vi "Process.vi"(8 "error in":errorcluster, 11 "Generator":refnum<class "Generator.lvclass">) -> (0 "error out":errorcluster, 3 "Generator out":refnum<class "Generator.lvclass">)   [LabVIEW 2019, in "Generator.lvclass"]
uses:
  Generator.lvclass
  <vilib>/JKI/JKI SMO/SMO/SMO.lvclass
  <userlib>/LevyLab/Debug/Debug.lvlib
  typedefs/Generator.State--enum.ctl
  929f499e-e52d-49ce-8fd4-6eb7de19c2ac.vi
  9c9ff3dc-a17c-4e79-91bb-522cf085dd97.vi
  7f9fb2fb-b452-4165-b08b-fdce49342378.vi
  C:/Program Files/National Instruments/LabVIEW 2019/vi.lib/JKI/JKI SMO/SMO/SMO.lvclass
panel:
  out "time (ms)":dbl=1.0 min=1.0 format="%#_6p"
  out "String 3":string
  in  "timeout (ms)":i32=10 min=1
  out "String 2":string
  out "String":string
  # "Generator"
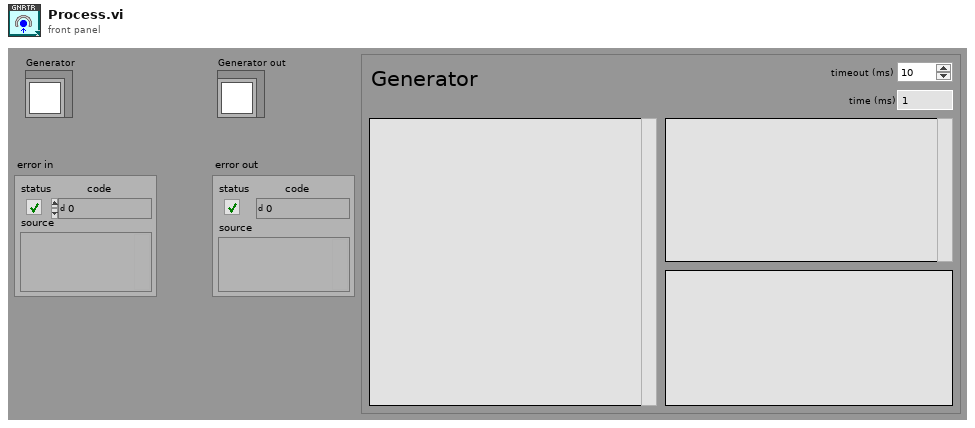
[diagram p1: front panel]
types:
  T1 = typedef "Generator.lvclass/Generator.State--enum.ctl" = enum16{"idle", "started"}
  T2 = enum32{"invalid app kind", "Development System", "Run Time System", "Student Edition", "Embedded LabVIEW", "Evaluation", "Custom"}
  T3 = enum32{"Invalid", "Standard", "Closed", "Hidden", "Minimized", "Maximized"}
  T4 = cluster{"Core":cluster{"Current VI Reference":refnum<vi>, "Close Panel on Exit?":bool, "Last Error":cluster{"error":errorcluster, "previous state":string, "remaining states":string}, "Shutdown?":bool}, "SelfRef":refnum<class "Generator.lvclass">, "state":T1}
  T5 = typedef "Generator.lvclass/AO.Channel--Cluster--Array.ctl" = T6[]
  T6 = typedef "Generator.lvclass/AO.Channel--Cluster.ctl" = cluster{"Enable?":bool, "Channel":i32, "Amplitude":dbl, "Offset":dbl, "Frequency":dbl, "Phase":dbl, "Function":T7, "Sweeping?":bool, "Limit AC?":bool, "Limit DC?":bool, "Duty Cycle?":bool, "Duty Cycle":dbl}
  T7 = typedef "Generator.lvclass/AO.Channel.Function--Enum.ctl" = enum16{"sine", "square", "triangle", "saw"}
  T8 = typedef "Generator.lvclass/REF.Channel--Cluster--Array.ctl" = T9[]
  T9 = typedef "Generator.lvclass/REF.Channel--Cluster.ctl" = cluster{"Enable?":bool, "Channel":i32, "Frequency":dbl, "Phase":dbl, "TC":dbl, "Roll-Off":i32}
  T10 = typedef "Generator.lvclass/Sweep.Channel--Cluster--Array.ctl" = T11[]
  T11 = typedef "Generator.lvclass/Sweep.Channel--Cluster.ctl" = cluster{"Enable?":bool, "Channel":u16, "Start":dbl, "End":dbl, "Pattern":T12, "Table":dbl[]}
  T12 = typedef "Generator.lvclass/Sweep.Pattern--Enum.ctl" = enum16{"Ramp /", "Ramp /\\", "Smooth Ramp _/", "Smooth Ramp _/\\_", "Table"}
  T13 = typedef "Generator.lvclass/Generator.Command--enum.ctl" = enum16{"start", "stop", "start sweep", "stop sweep"}
  T14 = cluster{"Current VI Reference":refnum<vi>, "Close Panel on Exit?":bool, "Last Error":cluster{"error":errorcluster, "previous state":string, "remaining states":string}, "Shutdown?":bool}
  T15 = typedef "Debug.lvlib/Attribute.Debug.lvclass/DebugBehavior.ctl" = enum16{"Normal", "Debug"}
  T16 = typedef "SMO.lvclass/Protected Events.ctl" = cluster{"StopProcesses":refnum<user-event>, "AbortProcesses":refnum<user-event>, "Config Changed":refnum<user-event>, "Dependency":refnum<user-event>}
  T17 = typedef "Generator.lvclass/PrivateEvents--Cluster.ctl" = cluster{"Message":refnum<user-event>, "Sampling":refnum<user-event>, "AOchannel":refnum<user-event>, "REFchannel":refnum<user-event>, "Sweep":refnum<user-event>, "Command":refnum<user-event>, "WaveformQueues":refnum<user-event>}
  T18 = typedef "Generator.lvclass/Waveforms--Cluster.ctl" = cluster{"AO":waveform(dbl)[], "REF_X":waveform(dbl)[], "REF_Y":waveform(dbl)[]}
  T19 = typedef "Generator.lvclass/Generator.Sweep Status--enum.ctl" = enum16{"idle", "initializing", "waiting", "sweeping", "stopping"}
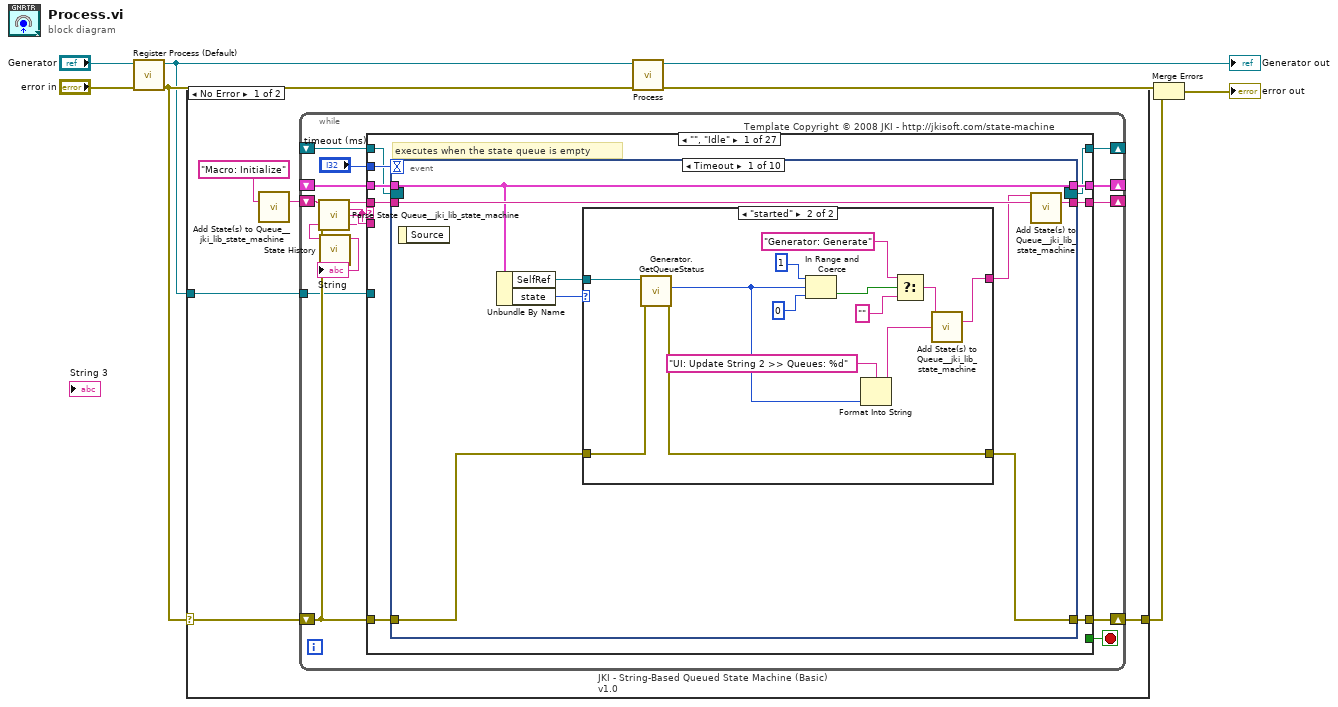
[diagram p0: block diagram]
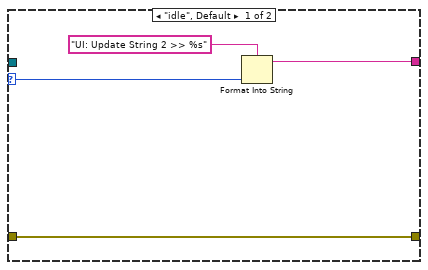
[diagram p2: hidden frame]
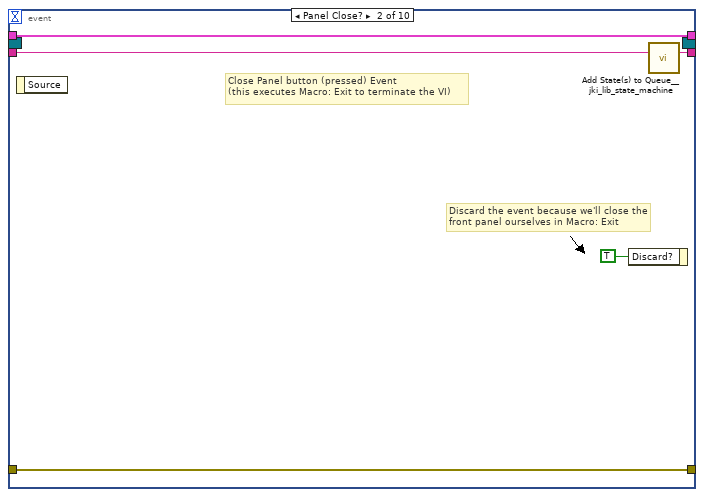
[diagram p3: hidden frame]
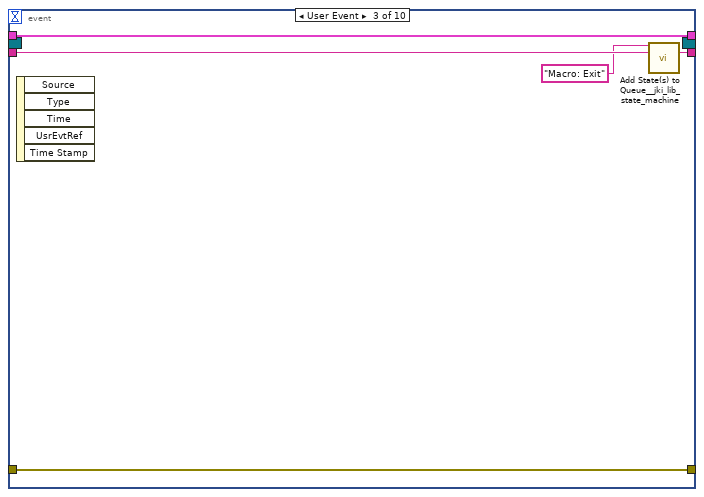
[diagram p4: hidden frame]
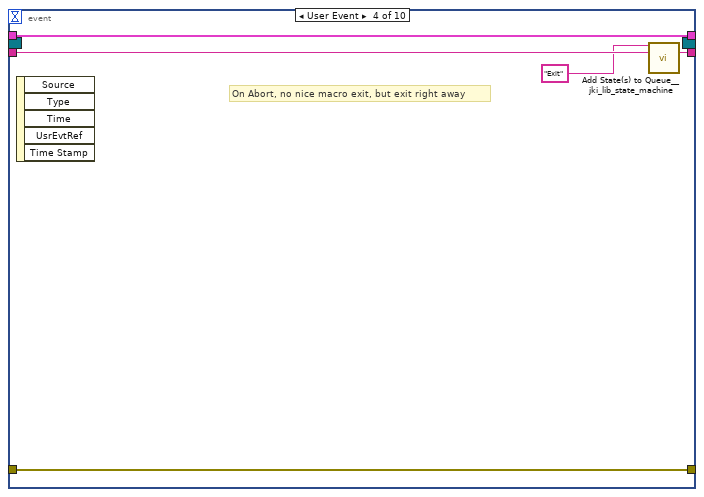
[diagram p5: hidden frame]
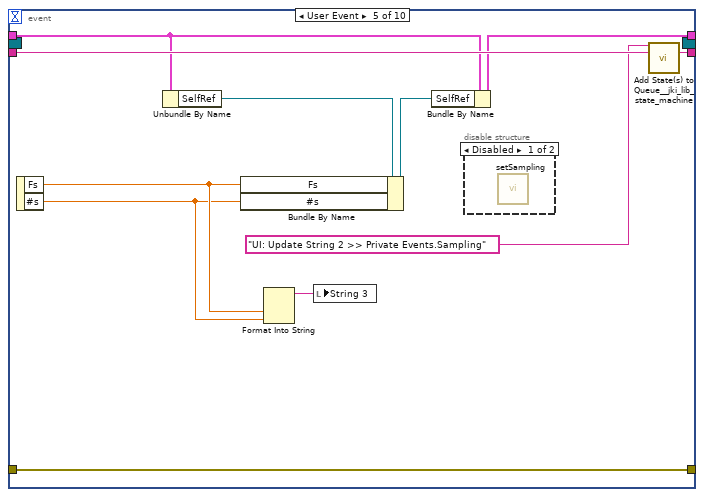
[diagram p6: hidden frame]
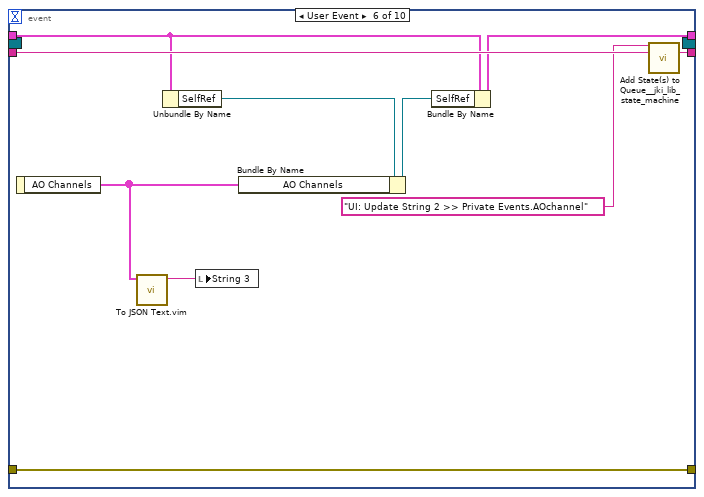
[diagram p8: hidden frame]
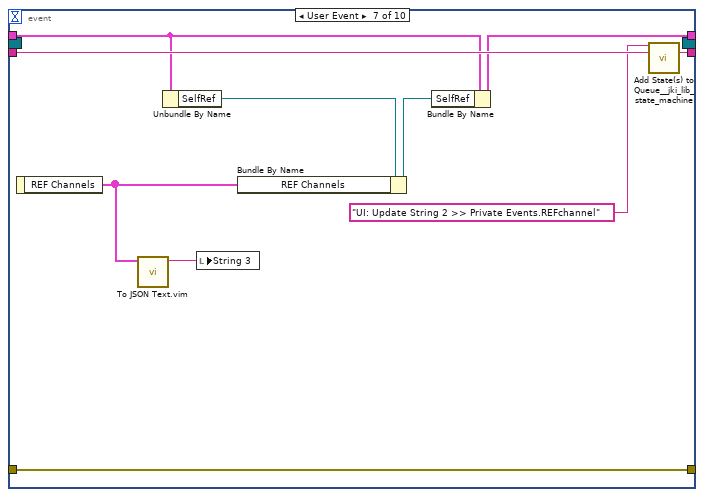
[diagram p9: hidden frame]
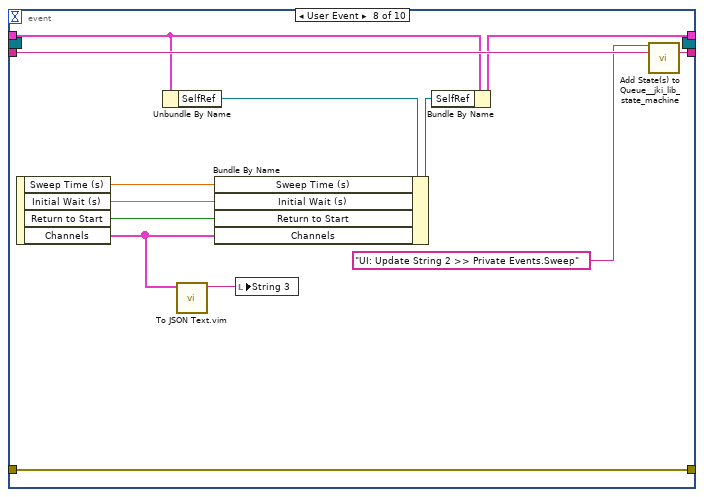
[diagram p10: hidden frame]
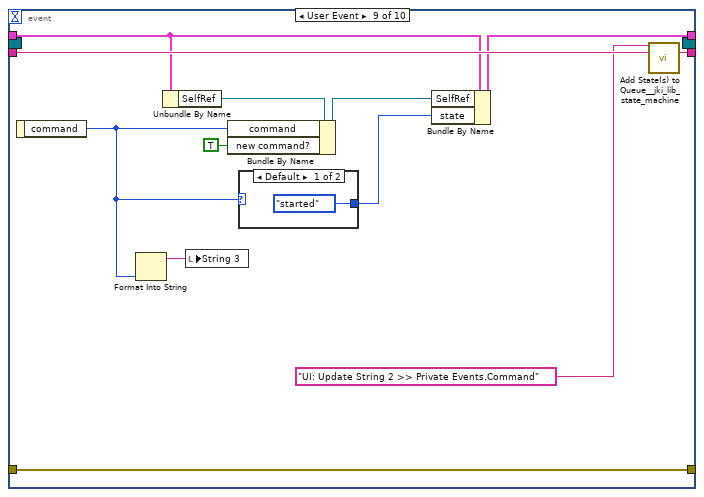
[diagram p11: hidden frame]
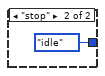
[diagram p12: hidden frame]
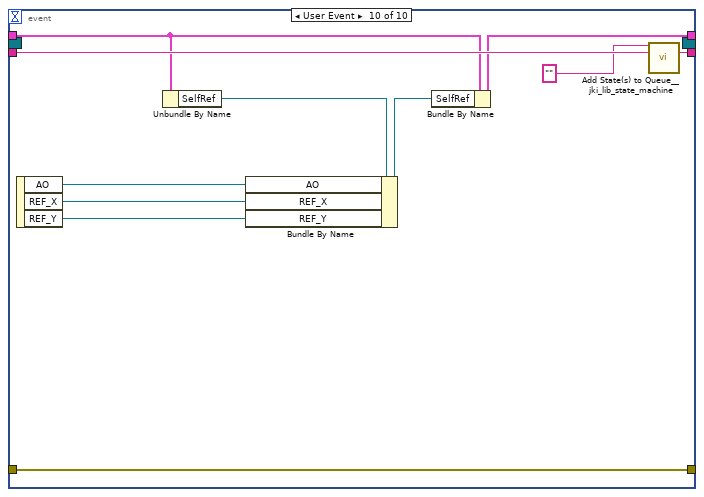
[diagram p13: hidden frame]
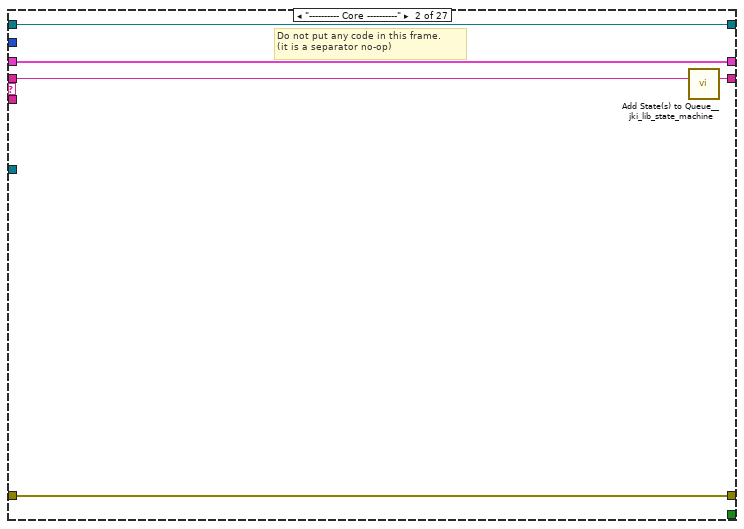
[diagram p14: hidden frame]
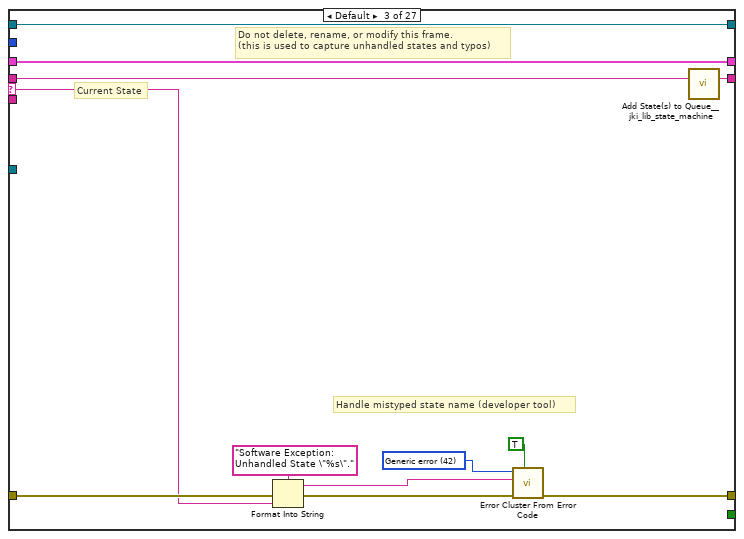
[diagram p15: hidden frame]
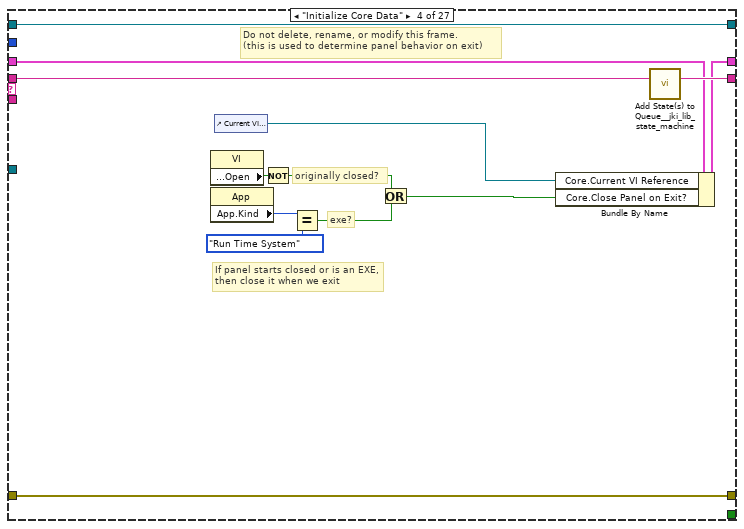
[diagram p16: hidden frame]
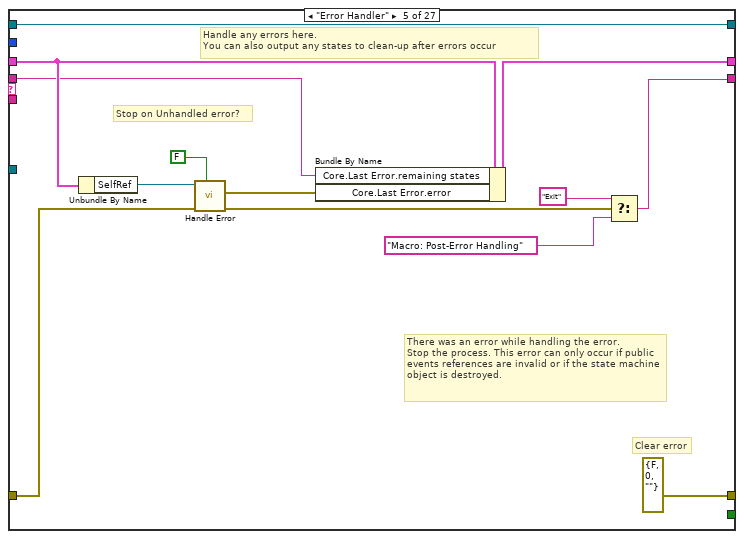
[diagram p17: hidden frame]
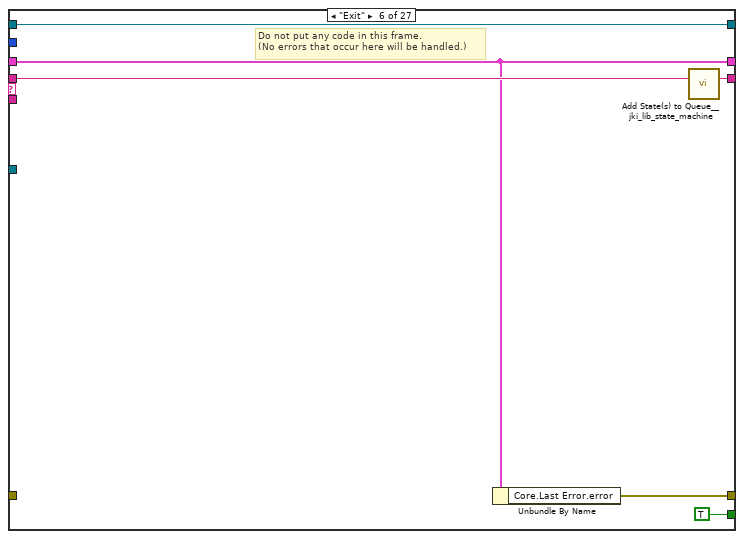
[diagram p18: hidden frame]
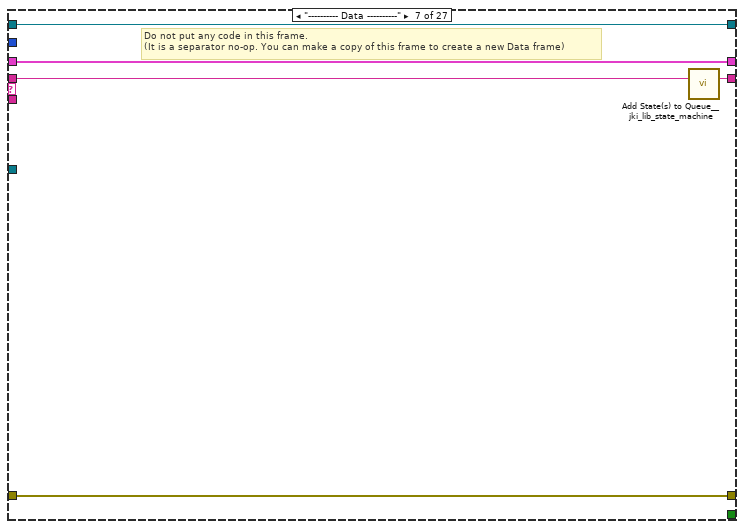
[diagram p19: hidden frame]
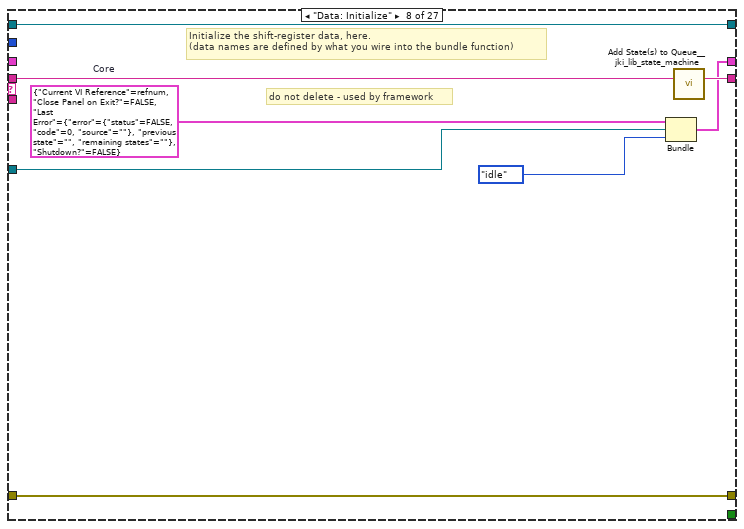
[diagram p20: hidden frame]
diagram:
  n1 = call <vilib>:"Register Process (Default).vi"("error in (no error)"="error in", "SMO"="Generator") -> ("error out"=w4:errorcluster, "SelfRef"=w3:refnum<class "Generator.lvclass">)  [unwired: 8 in]
  n2 = case shown="No Error" w4 {
    selector: w4 -> [w12 w440]
    tunnel: w3 -> [w13 _]
    tunnel: [w11 w440] -> w2
    frame No Error {
      n3 = call <vilib>:"Add State(s) to Queue__jki_lib_state_machine.vi"("State(s) in (\"\")"="Macro: Initialize") -> ("States Out"=w9:string)  [unwired: 14 in]
      n4 = while "JKI - String-Based Queued State Machine (Basic) v1.0" {
        shift-right: [w22] -> _
        shift-left: _ -> [w21]
        shift-right: [w25] -> w11
        shift-left: w12 -> [w20]
        shift-right: [w24] -> _
        shift-left: w9 -> [w26]
        tunnel: w13 -> [w19]
        shift-right: [w18] -> _
        shift-left: _ -> [w17]
        stop <- w23 stop-if-true
        # "Template Copyright © 2008 JKI - http://jkisoft.com/state-machine"
        n5 = call <vilib>:"Parse State Queue__jki_lib_state_machine.vi"("State Queue"=w26, "Error In (no error)"=w20) -> ("Remaining States"=w28:string, "Current State"=w16:string, "Arguments"=w27:string)  [unwired: 11 in]
        n6 = call "State History.vi"("Current State"=w16) -> ("History"=→"String":string)  [unwired: 10 in]
        n7 = case shown="\"\", \"Idle\"" w16 {
          selector: w16 -> [_ _ w153 _ _ _ _ _ _ _ _ _ w237 _ _ _ _ _ _ _ _ _ _ _ _ _ _]
          tunnel: w28 -> [w37 w151 w157 w176 w178 w195 w200 w208 w215 w220 w226 w233 w236 w256 w272 w304 w313 w319 w345 w362 w367 w378 w383 w396 w402 w409 w429]
          tunnel: w27 -> [_ _ _ _ _ _ _ _ _ _ _ w227 w234 w250 w268 _ _ _ _ _ _ _ _ _ _ _ _]
          tunnel: w21 -> [w35 w148 w155 w167 w187 w191 w197 _ w210 w217 w224 w230 w247 w254 w270 w301 w309 w316 w337 w352 w364 w375 w380 w394 w400 w405 w422]
          tunnel: [w34 w149 w159 w173 errorcluster {"status"=FALSE, "code"=0, "source"=""} ("error out") w190 w198 w203 w211 w218 w222 w231 w248 w251 w265 w302 w311 w315 w343 w360 w365 w369 w381 w387 w398 w403 w423] -> w25
          tunnel: w20 -> [w33 w149 w158 w173 w184 _ w198 w203 w212 w218 w221 w231 w248 w252 w266 w302 w311 w314 w343 w360 w365 w370 w381 w390 w398 w403 w425]
          tunnel: [w36 w150 w156 w175 w177 w194 w199 w207 w214 w219 w225 w232 w249 w255 w271 w303 w312 w328 w344 w361 w366 w377 w382 w395 w401 w408 w428] -> w24
          tunnel: [_ _ _ _ _ TRUE _ _ _ _ _ _ _ _ _ _ _ _ _ _ _ _ _ _ _ _ _] -> w23
          tunnel: [w32 w148 w155 w174 w186 w191 w197 w206 w210 w217 w224 w230 w247 w254 w270 w301 w309 w317 w341 w351 w364 w375 w380 w394 w400 w406 w426] -> w22
          tunnel: "timeout (ms)" -> [w31 _ _ _ _ _ _ _ _ _ _ _ _ _ _ _ _ _ _ _ _ _ _ _ _ _ _]
          tunnel: w19 -> [_ _ _ _ _ _ _ w202 _ _ _ _ _ _ _ _ _ _ _ _ _ _ _ _ _ _ _]
          tunnel: [w29 w147 w152 w164 w189 w192 w196 w205 w209 w216 w223 w229 w246 w253 w269 w300 w310 w327 w342 w354 w363 w376 w379 w392 w399 w407 w427] -> w18
          tunnel: w17 -> [w30 w147 w152 w164 w189 w192 w196 w205 w209 w216 w223 w229 w246 w253 w269 w300 w310 w327 w342 w354 w363 w376 w379 _ w399 w407 w427]
          frame "", "Idle" {
            # "executes when the state queue is empty"
            n8 = event shown="[0] Timeout" {
              selector: w30 -> [_ _ _ _ _ _ _ _ _ _]
              dyn-events: [_ _ _ _ _ _ _ _ _ _] -> w29
              timeout: w31 -> [_ _ _ _ _ _ _ _ _ _]
              tunnel: w37 -> [w45 w67 w72 w77 w88 w98 w108 w121 w133 w146]
              tunnel: [w44 w66 w71 w76 w87 w97 w107 w120 w132 w145] -> w36
              tunnel: w35 -> [w43 w63 w69 w74 w82 w91 w102 w113 w126 w138]
              tunnel: [w39 w65 w70 w75 w86 w96 w106 w119 w131 w144] -> w34
              tunnel: w33 -> [w40 w65 w70 w75 w86 w96 w106 w119 w131 w144]
              tunnel: [w43 w63 w69 w74 w83 w92 w103 w114 w127 w139] -> w32
              event Timeout {
                n9 = event-data() -> ()  [unwired: 1 in, 1 out]
                n10 = Unbundle By Name(w43) -> ("SelfRef"=w42:refnum<class "Generator.lvclass">, "state"=w38:T1)
                n11 = case shown="\"started\"" w38 {
                  selector: w38 -> [w48 _]
                  tunnel: w42 -> [_ w62]
                  tunnel: [w46 w51] -> w41
                  tunnel: w40 -> [w49 w55]
                  tunnel: [w49 w54] -> w39
                  frame "idle", Default {
                    n12 = Format Into String(format string="UI: Update String 2 >> %s" ("f"), w48) -> (resulting string=w46:string)  [unwired: 2 in, 1 out]
                  }
                  frame "started" {
                    n13 = call "Generator.GetQueueStatus.vi"("error in (no error)"=w55, "Generator in"=w62) -> ("error out"=w54:errorcluster, "# elements"=w59:i32)  [unwired: 7 in, 1 out]
                    n14 = In Range and Coerce(upper limit=1 ("x"), x=w59, lower limit=0 ("x")) -> (In Range?=w58:bool)  [unwired: 1 out]
                    n15 = Format Into String(format string="UI: Update String 2 >> Queues: %d" ("f"), w59) -> (resulting string=w53:string)  [unwired: 2 in, 1 out]
                    n16 = Select(t="Generator: Generate", s=w58, f="") -> (s? t:f=w52:string)
                    n17 = call <vilib>:"Add State(s) to Queue__jki_lib_state_machine.vi"("State(s) in Front (\"\")"=w52, "State(s) at Back (\"\")"=w53) -> ("States Out"=w51:string)  [unwired: 13 in]
                  }
                }
                n18 = call <vilib>:"Add State(s) to Queue__jki_lib_state_machine.vi"("State(s) in Front (\"\")"=w41, "State(s) in (\"\")"=w45) -> ("States Out"=w44:string)  [unwired: 13 in]
              }
              event Panel Close? {
                # "Discard the event because we'll close the front panel ourselves in Macro: Exit"
                # "Close Panel button (pressed) Event\n(this executes Macro: Exit to terminate the VI)"
                n19 = event-data() -> ()  [unwired: 1 in, 1 out]
                n20 = event-data("Discard?"=TRUE) -> ()  [unwired: 1 in, 1 out]
                n21 = call <vilib>:"Add State(s) to Queue__jki_lib_state_machine.vi"("State(s) in (\"\")"=w67) -> ("States Out"=w66:string)  [unwired: 14 in]
              }
              event User Event {
                n22 = event-data() -> ()  [unwired: 1 in, 5 out]
                n23 = call <vilib>:"Add State(s) to Queue__jki_lib_state_machine.vi"("State(s) in Front (\"\")"="Macro: Exit", "State(s) in (\"\")"=w72) -> ("States Out"=w71:string)  [unwired: 13 in]
              }
              event User Event {
                # "On Abort, no nice macro exit, but exit right away"
                n24 = event-data() -> ()  [unwired: 1 in, 5 out]
                n25 = call <vilib>:"Add State(s) to Queue__jki_lib_state_machine.vi"("State(s) in Front (\"\")"="Exit", "State(s) in (\"\")"=w77) -> ("States Out"=w76:string)  [unwired: 13 in]
              }
              event User Event {
                n26 = event-data() -> ("Fs"=w79:dbl, "#s"=w78:dbl)  [unwired: 1 in]
                n27 = Unbundle By Name(w82) -> ("SelfRef"=w85:refnum<class "Generator.lvclass">)
                n28 = Bundle By Name(cluster=w85, "Fs"=w79, "#s"=w78) -> (w84:refnum<class "Generator.lvclass">)
                n29 = Format Into String(w79, w78) -> (resulting string=w80:string)  [unwired: 3 in, 1 out]
                n30 = local write "String 3"(w80) -> ()
                n31 = Bundle By Name(cluster=w82, "SelfRef"=w84) -> (w83:T4)
                n32 = disable-structure shown="Disabled" {
                  frame Disabled {
                    n33 = call "setSampling.vi"() -> ()  [unwired: 10 in, 2 out]
                  }
                  frame Enabled {
                  }
                }
                n34 = call <vilib>:"Add State(s) to Queue__jki_lib_state_machine.vi"("State(s) in Front (\"\")"="UI: Update String 2 >> Private Events.Sampling", "State(s) in (\"\")"=w88) -> ("States Out"=w87:string)  [unwired: 13 in]
              }
              event User Event {
                n35 = event-data() -> ("AO Channels"=w90:T5)  [unwired: 1 in]
                n36 = call "To JSON Text.vim"("Anything"=w90) -> ("<JSON>"=w89:string)  [unwired: 9 in, 1 out]
                n37 = Unbundle By Name(w91) -> ("SelfRef"=w94:refnum<class "Generator.lvclass">)
                n38 = local write "String 3"(w89) -> ()
                n39 = Bundle By Name(cluster=w94, "AO Channels"=w90) -> (w93:refnum<class "Generator.lvclass">)
                n40 = Bundle By Name(cluster=w91, "SelfRef"=w93) -> (w92:T4)
                n41 = call <vilib>:"Add State(s) to Queue__jki_lib_state_machine.vi"("State(s) in Front (\"\")"="UI: Update String 2 >> Private Events.AOchannel", "State(s) in (\"\")"=w98) -> ("States Out"=w97:string)  [unwired: 13 in]
              }
              event User Event {
                n42 = event-data() -> ("REF Channels"=w99:T8)  [unwired: 1 in]
                n43 = call "To JSON Text.vim"("Anything"=w99) -> ("<JSON>"=w100:string)  [unwired: 9 in, 1 out]
                n44 = Unbundle By Name(w102) -> ("SelfRef"=w105:refnum<class "Generator.lvclass">)
                n45 = local write "String 3"(w100) -> ()
                n46 = Bundle By Name(cluster=w105, "REF Channels"=w99) -> (w104:refnum<class "Generator.lvclass">)
                n47 = Bundle By Name(cluster=w102, "SelfRef"=w104) -> (w103:T4)
                n48 = call <vilib>:"Add State(s) to Queue__jki_lib_state_machine.vi"("State(s) in Front (\"\")"="UI: Update String 2 >> Private Events.REFchannel", "State(s) in (\"\")"=w108) -> ("States Out"=w107:string)  [unwired: 13 in]
              }
              event User Event {
                n49 = event-data() -> ("Sweep Time (s)"=w117:dbl, "Initial Wait (s)"=w111:dbl, "Return to Start"=w112:bool, "Channels"=w109:T10)  [unwired: 1 in]
                n50 = Unbundle By Name(w113) -> ("SelfRef"=w116:refnum<class "Generator.lvclass">)
                n51 = call "To JSON Text.vim"("Anything"=w109) -> ("<JSON>"=w110:string)  [unwired: 9 in, 1 out]
                n52 = Bundle By Name(cluster=w116, "Sweep Time (s)"=w117, "Initial Wait (s)"=w111, "Return to Start"=w112, "Channels"=w109) -> (w115:refnum<class "Generator.lvclass">)
                n53 = local write "String 3"(w110) -> ()
                n54 = Bundle By Name(cluster=w113, "SelfRef"=w115) -> (w114:T4)
                n55 = call <vilib>:"Add State(s) to Queue__jki_lib_state_machine.vi"("State(s) in Front (\"\")"="UI: Update String 2 >> Private Events.Sweep", "State(s) in (\"\")"=w121) -> ("States Out"=w120:string)  [unwired: 13 in]
              }
              event User Event {
                n56 = event-data() -> ("command"=w123:T13)  [unwired: 1 in]
                n57 = Format Into String(w123) -> (resulting string=w124:string)  [unwired: 3 in, 1 out]
                n58 = Unbundle By Name(w126) -> ("SelfRef"=w129:refnum<class "Generator.lvclass">)
                n59 = local write "String 3"(w124) -> ()
                n60 = Bundle By Name(cluster=w129, "command"=w123, "new command?"=TRUE) -> (w128:refnum<class "Generator.lvclass">)
                n61 = case shown="Default" w123 {
                  tunnel: [Generator.State--enum."started" ("state") Generator.State--enum."idle" ("state")] -> w125
                  frame Default {
                  }
                  frame "stop" {
                  }
                }
                n62 = Bundle By Name(cluster=w126, "SelfRef"=w128, "state"=w125) -> (w127:T4)
                n63 = call <vilib>:"Add State(s) to Queue__jki_lib_state_machine.vi"("State(s) in Front (\"\")"="UI: Update String 2 >> Private Events.Command", "State(s) in (\"\")"=w133) -> ("States Out"=w132:string)  [unwired: 13 in]
              }
              event User Event {
                n64 = event-data() -> ("AO"=w142:refnum<queue>, "REF_X"=w137:refnum<queue>, "REF_Y"=w136:refnum<queue>)  [unwired: 1 in]
                n65 = Unbundle By Name(w138) -> ("SelfRef"=w141:refnum<class "Generator.lvclass">)
                n66 = Bundle By Name(cluster=w141, "AO"=w142, "REF_X"=w137, "REF_Y"=w136) -> (w140:refnum<class "Generator.lvclass">)
                n67 = Bundle By Name(cluster=w138, "SelfRef"=w140) -> (w139:T4)
                n68 = call <vilib>:"Add State(s) to Queue__jki_lib_state_machine.vi"("State(s) in Front (\"\")"="", "State(s) in (\"\")"=w146) -> ("States Out"=w145:string)  [unwired: 13 in]
              }
            }
          }
          frame "---------- Core ----------" {
            # "Do not put any code in this frame.\n(it is a separator no-op)"
            n69 = call <vilib>:"Add State(s) to Queue__jki_lib_state_machine.vi"("State(s) in (\"\")"=w151) -> ("States Out"=w150:string)  [unwired: 14 in]
          }
          frame Default {
            w162 = 42 items=["No error", "Argument error", "Memory is full", "Out of zone", "End of file", "File already open", "Generic file I/O error", "File not found", "File permission error", "Disk is full", "Duplicate path", "Too many files open", "System feature not enabled", "Resource file not found", "Cannot add resource", "Resource not found", "Image not found", "Image memory error", "Pen does not exist", "Config type invalid", "Config token not found", "Config parse error", "Config memory error", "Bad external code format", "Bad external code offset", "External code not present", "Null window", "Destroy window error", "Null menu", "Print aborted", "Bad print record", "Print driver error", "Windows error during printing", "Memory error during printing", "Print dialog error", "Generic print error", "Invalid device refnum", "Device not found", "Device parameter error", "Device unit error", "Cannot open device", "Device call aborted", "Generic error", "Cancelled by user", "Object ID too low", "Object ID too high", "Object not in heap", "Unknown heap", "Unknown object (invalid DefProc)", "Unknown object (DefProc not in table)", "Message out of range", "Invalid (null) method", "Unknown message", "Manager call not supported", "Bad address", "Network operation in progress", "Network operation timed out", "Connection is busy", "Network attribute not supported", "Network error", "Address in use", "System out of memory", "Connection aborted", "Connection refused", "Not connected", "Already connected", "Connection closed", "Initialization error (interapplication manager)", "Bad occurrence", "Wait on unbound occurrence handler", "Occurrence queue overflow", "Datalog type conflict", "Unused", "Unrecognized type (interapplication manager)", "Memory corrupt", "Failed to make temporary DLL", "Old CIN version", "Drag socket not found", "Failed to load drop-object", "Failed to register OLE object", "Failed to release OLE object", "Format specifier type mismatch", "Unknown format specifier", "Too few format specifiers", "Too many format specifiers", "Scan failed", "Newer CIN version", "Error converting to variant", "Runtime menu error", "Password tampered", "Variant attribute not found", "Incompatible variant data type", "Event data is not available", "Event Store is not present", "Occurrence is not found", "Event Queue is not created", "Event info is not available", "Refnum passed is NULL", "Error retrieving Class GUID", "Error retrieving CoClass GUID", "Error retrieving TypeLib GUID.", "Bad built application magic bytes.", "Specific driver is different from the specific driver associated with the Logical Name.", "There is no session opened to the class driver.", "Max Error", "MAX - Error with config objects", "MAX - Error loading configuration", "MAX - Group not supported"]
            # "Current State"
            # "Do not delete, rename, or modify this frame.\n(this is used to capture unhandled states and typos)"
            # "Handle mistyped state name (developer tool)"
            n70 = Format Into String(format string="Software Exception: Unhandled State \"%s\"." ("message"), error in=w158, w153) -> (resulting string=w161:string, error out=w160:errorcluster)  [unwired: 1 in]
            n71 = call <vilib>:"Error Cluster From Error Code.vi"("show call chain? (False)"=TRUE, "error in (no error)"=w160, "error message (\"\")"=w161, "error code (0)"=w162) -> ("error out"=w159:errorcluster)  [unwired: 5 in]
            n72 = call <vilib>:"Add State(s) to Queue__jki_lib_state_machine.vi"("State(s) in (\"\")"=w157) -> ("States Out"=w156:string)  [unwired: 14 in]
          }
          frame "Initialize Core Data" {
            # "Do not delete, rename, or modify this frame.\n(this is used to determine panel behavior on exit)"
            # "originally closed?"
            # "exe?"
            # "If panel starts closed or is an EXE, then close it when we exit"
            n73 = property class="VI"() -> ("Front Panel.Open"=w172:bool)  [unwired: 2 in, 2 out]
            n74 = property class="App"() -> ("App.Kind"=w171:T2)  [unwired: 2 in, 2 out]
            n75 = control-ref of="Current VI Reference"() -> (w165:refnum<vi>)
            n76 = Not(x=w172) -> (.not. x?=w169:bool)
            n77 = Equal?(x=w171, y=T2."Run Time System" ("Application:Kind")) -> (x = y?=w168:bool)
            n78 = Or(x=w169, y=w168) -> (x .or. y?=w166:bool)
            n79 = Bundle By Name(cluster=w167, "Core.Current VI Reference"=w165, "Core.Close Panel on Exit?"=w166) -> (w174:T4)
            n80 = call <vilib>:"Add State(s) to Queue__jki_lib_state_machine.vi"("State(s) in (\"\")"=w176) -> ("States Out"=w175:string)  [unwired: 14 in]
          }
          frame "Error Handler" {
            # "Stop on Unhandled error?"
            # "There was an error while handling the error.\nStop the process. This error can only occur if public events references are invalid or if the state machine object is destroyed."
            # "Handle any errors here.\nYou can also output any states to clean-up after errors occur"
            # "Clear error"
            n81 = Unbundle By Name(w187) -> ("SelfRef"=w188:refnum<class "Generator.lvclass">)
            n82 = call-dynamic "Handle Error.vi"("Stop on Unhandled Error (T)"=FALSE, "error in"=w184, "SMO"=w188) -> ("handling error"=w182:errorcluster, "Unhandled error"=w185:errorcluster)  [unwired: 6 in, 1 out]
            n83 = Bundle By Name(cluster=w187, "Core.Last Error.remaining states"=w178, "Core.Last Error.error"=w185) -> (w186:T4)
            n84 = Select(t="Exit", s=w182, f="Macro: Post-Error Handling") -> (s? t:f=w177:string)
          }
          frame "Exit" {
            # "Do not put any code in this frame.\n(No errors that occur here will be handled.)"
            n85 = Unbundle By Name(w191) -> ("Core.Last Error.error"=w190:errorcluster)
            n86 = call <vilib>:"Add State(s) to Queue__jki_lib_state_machine.vi"("State(s) in (\"\")"=w195) -> ("States Out"=w194:string)  [unwired: 14 in]
          }
          frame "---------- Data ----------" {
            # "Do not put any code in this frame.\n(It is a separator no-op. You can make a copy of this frame to create a new Data frame)"
            n87 = call <vilib>:"Add State(s) to Queue__jki_lib_state_machine.vi"("State(s) in (\"\")"=w200) -> ("States Out"=w199:string)  [unwired: 14 in]
          }
          frame "Data: Initialize" {
            w204 = T14 {"Current VI Reference"=refnum, "Close Panel on Exit?"=FALSE, "Last Error"={"error"={"status"=FALSE, "code"=0, "source"=""}, "previous state"="", "remaining states"=""}, "Shutdown?"=FALSE}  # Core
            # "do not delete - used by framework"
            # "Initialize the shift-register data, here.\n(data names are defined by what you wire into the bundle function)"
            n88 = Bundle("Core"=w204, "SelfRef"=w202, "state"=Generator.State--enum."idle") -> (w206:T4)  [unwired: 1 in]
            n89 = call <vilib>:"Add State(s) to Queue__jki_lib_state_machine.vi"("State(s) in (\"\")"=w208) -> ("States Out"=w207:string)  [unwired: 14 in]
          }
          frame "Data: Cleanup" {
            # "Cleanup any data and references, here.\n(this is called automatically, by the Macro: Exit)"
            n90 = Unbundle By Name(w210) -> ("Core.Current VI Reference"=w213:refnum<vi>)
            n91 = Close Reference(reference=w213, error in (no error)=w212) -> (error out=w211:errorcluster)
            n92 = call <vilib>:"Add State(s) to Queue__jki_lib_state_machine.vi"("State(s) in (\"\")"=w215) -> ("States Out"=w214:string)  [unwired: 14 in]
          }
          frame "---------- UI ----------" {
            # "Do not put any code in this frame.\n(It is a separator no-op. You can make a copy of this frame to create a new UI frame)"
            n93 = call <vilib>:"Add State(s) to Queue__jki_lib_state_machine.vi"("State(s) in (\"\")"=w220) -> ("States Out"=w219:string)  [unwired: 14 in]
          }
          frame "UI: Initialize" {
            # "Initialize the User Interface, here.\n(this is called automatically, by the Macro: Init)"
            n94 = flat-sequence {
              frame #0 {
                # "This is to keep in memory\nfor EXE build"
              }
            }
            n95 = call <userlib>:"Fit VI window to Largest Dec__ogtk.vi"("error in (no error)"=w221) -> ("error out"=w222:errorcluster)  [unwired: 5 in, 1 out]
            n96 = call <vilib>:"Add State(s) to Queue__jki_lib_state_machine.vi"("State(s) in (\"\")"=w226) -> ("States Out"=w225:string)  [unwired: 14 in]
          }
          frame "UI: Update String 2" {
            # "Do not put any code in this frame.\n(It is a separator no-op. You can make a copy of this frame to create a new UI frame)"
            n97 = call "State History.vi"("Current State"=w227) -> ("History"=→"String 2":string)  [unwired: 10 in]
            n98 = call <vilib>:"Add State(s) to Queue__jki_lib_state_machine.vi"("State(s) in (\"\")"=w233) -> ("States Out"=w232:string)  [unwired: 14 in]
          }
          frame "UI: Wait" {
            # "UI: Wait.\n(use: \"UI: Wait >> time\" (in ms))"
            n99 = Scan From String(format string="%d", input string=w234, default 1=u32 0 ("default value 1")) -> (output 1=w243:u32)  [unwired: 2 in, 3 out]
            n100 = feedback #1(TRUE ("Triggered")) -> (w240:bool)
            n101 = call <userlib>:"Periodic Trigger__ogtk.vi"("time (ms)"=w243, "reset"=w240) -> ("Triggered"=w241:bool)  [unwired: 11 in, 2 out]
            n102 = feedback-in #1(w241) -> ()
            n103 = call <vilib>:"Build State String with Arguments__JKI_lib_State_Machine.vi"("Arguments (\"\")"=w234, "State"=w237) -> ("State with Arguments"=w239:string)  [unwired: 4 in]
            n104 = Select(t="", s=w241, f=w239) -> (s? t:f=w235:string)
            n105 = call <vilib>:"Add State(s) to Queue__jki_lib_state_machine.vi"("State(s) in Front (\"\")"=w235, "State(s) in (\"\")"=w236) -> ("States Out"=w249:string)  [unwired: 13 in]
          }
          frame "UI: Cursor Set" {
            # "Argument"
            # "Initialize the User Interface, here.\n(this is called automatically, by the Macro: Init)"
            n106 = disable-structure shown="Default" {
              disable-tunnel: w252 -> [w257 w260]
              disable-tunnel: [w257 w259] -> w251
              disable-tunnel: w250 -> [_ w258]
              frame condition #0 {
              }
              frame condition #1 (active) {
                n107 = case shown="\"Idle\", Default" w258 {
                  tunnel: w260 -> [w262 w264]
                  tunnel: [w261 w263] -> w259
                  frame "Idle", Default {
                    n108 = call <vilib>:"Unset Busy.vi"("error in (no error)"=w262) -> ("error out"=w261:errorcluster)  [unwired: 10 in]
                  }
                  frame "Busy" {
                    n109 = call <vilib>:"Set Busy.vi"("error in (no error)"=w264) -> ("error out"=w263:errorcluster)  [unwired: 9 in, 1 out]
                  }
                }
              }
            }
            n110 = call <vilib>:"Add State(s) to Queue__jki_lib_state_machine.vi"("State(s) in (\"\")"=w256) -> ("States Out"=w255:string)  [unwired: 14 in]
          }
          frame "UI: Front Panel State" {
            # "Argument"
            # "Set Front Panel Open or Closed\n(Usage: \"UI: Front Panel State >> Open|Close\")"
            n111 = Unbundle By Name(w270) -> ("Core.Current VI Reference"=w267:refnum<vi>)
            n112 = disable-structure shown="Default" {
              disable-tunnel: w266 -> [w276 w299]
              disable-tunnel: [w275 w299] -> w265
              disable-tunnel: w267 -> [w274 _]
              disable-tunnel: w268 -> [w273 _]
              frame condition #0 (active) {
                n113 = case shown="\"Open\"" w273 {
                  tunnel: w276 -> [w280 w293]
                  tunnel: [w282 w294] -> w275
                  tunnel: w274 -> [w281 w291]
                  frame "Open" {
                    # "Open FP if not open or invalid"
                    n114 = property class="VI"(reference=w281, error in=w280) -> (reference out=w278:refnum<vi>, error out=w279:errorcluster, "FP.State"=w277:T3)
                    n115 = case shown="Default" w277 {
                      tunnel: [w285 w288] -> w282
                      tunnel: w279 -> [w284 w288]
                      tunnel: w278 -> [w283 _]
                      frame Default {
                        n116 = invoke class="VI" method="FP.Open"(reference=w283, error in=w284, "Activate"=TRUE, "State"=T3."Standard") -> (error out=w285:errorcluster)  [unwired: 1 in, 4 out]
                      }
                      frame "Invalid", "Standard" {
                      }
                    }
                  }
                  frame "Close", Default {
                    # "Close FP is not Closed or Invalid"
                    n117 = property class="VI"(reference=w291, error in=w293) -> (reference out=w290:refnum<vi>, error out=w292:errorcluster, "FP.State"=w289:T3)
                    n118 = case shown="Default" w289 {
                      tunnel: [w295 w298] -> w294
                      tunnel: w292 -> [w295 w297]
                      tunnel: w290 -> [_ w296]
                      frame "Invalid", "Closed" {
                      }
                      frame Default {
                        n119 = invoke class="VI" method="FP.Close"(reference=w296, error in=w297) -> (error out=w298:errorcluster)  [unwired: 1 in, 2 out]
                      }
                    }
                  }
                }
              }
              frame condition #1 {
              }
            }
            n120 = call <vilib>:"Add State(s) to Queue__jki_lib_state_machine.vi"("State(s) in (\"\")"=w272) -> ("States Out"=w271:string)  [unwired: 14 in]
          }
          frame "---------- Macro ----------" {
            # "Do not put any code in this frame.\n(It is a separator no-op. You can make a copy of this frame to create a new Macro frame)"
            n121 = call <vilib>:"Add State(s) to Queue__jki_lib_state_machine.vi"("State(s) in (\"\")"=w304) -> ("States Out"=w303:string)  [unwired: 14 in]
          }
          frame "Macro: Initialize" {
            w307 = "UI: Initialize\nUI: Front Panel State >> Close\nMacro: Debug"  # UI: Initialize UI: Front Panel State >> Close Macro: Debug
            # "Initialization Macro\n(This is called once, when the VI starts)"
            n122 = call <vilib>:"Add State(s) to Queue__jki_lib_state_machine.vi"("State(s) in Front (\"\")"="Data: Initialize\nInitialize Core Data\nEvents: Register", "State(s) in (\"\")"="Process: Sync", "State(s) at Back (\"\")"=w307) -> ("States Out"=w306:string)  [unwired: 12 in]
            n123 = call <vilib>:"Add State(s) to Queue__jki_lib_state_machine.vi"("State(s) in Front (\"\")"=w306, "State(s) in (\"\")"=w313) -> ("States Out"=w312:string)  [unwired: 13 in]
          }
          frame "Macro: Debug" {
            # "exe?"
            # "If pane is an EXE, then close it when we exit"
            # "Macro: Debug\n(get debug behavior, determine UI and determine shutdown behavior)"
            n124 = Unbundle By Name(w316) -> ("Core.Close Panel on Exit?"=w321:bool, "SelfRef"=w326:refnum<class "Generator.lvclass">)
            n125 = property class="App"() -> ("App.Kind"=w324:T2)  [unwired: 2 in, 2 out]
            n126 = Equal?(x=w324, y=T2."Run Time System" ("Application:Kind")) -> (x = y?=w320:bool)
            n127 = call <userlib>:"Get Debug Mode.vi"("error in (no error)"=w314, "SMO"=w326) -> ("error out"=w315:errorcluster, "Behavior"=w325:T15)  [unwired: 7 in, 1 out]
            n128 = case shown="\"Normal\", Default" w325 {
              tunnel: [w329 w331] -> w322
              tunnel: w321 -> [w329 _]
              tunnel: w320 -> [_ w333]
              tunnel: [_ "UI: Front Panel State >> Open\nUI: Wait >> 1000"] -> w318
              frame "Normal", Default {
                # "respect core.close"
              }
              frame "Debug" {
                # "keep panel open\nunless exe"
                n129 = Or(x=w333, y=FALSE) -> (x .or. y?=w331:bool)
              }
            }
            n130 = Bundle By Name(cluster=w316, "Core.Close Panel on Exit?"=w322) -> (w317:T4)
            n131 = call <vilib>:"Add State(s) to Queue__jki_lib_state_machine.vi"("State(s) in Front (\"\")"=w318, "State(s) in (\"\")"=w319) -> ("States Out"=w328:string)  [unwired: 13 in]
          }
          frame "Macro: Post-Error Handling" {
            # "Clear Last Error?"
            n132 = Unbundle By Name(w337) -> ("Core.Last Error.remaining states"=w335:string, "Core.Shutdown?"=w336:bool)
            n133 = Unbundle By Name(w337) -> ("Core.Last Error.error"=w340:errorcluster)
            n134 = case shown="False" FALSE {
              tunnel: w340 -> [w349 _]
              tunnel: [w349 _] -> w339
              frame False {
              }
              frame True {
              }
            }
            n135 = case shown="True" w336 {
              tunnel: w335 -> [w346 w348]
              tunnel: [w346 w347] -> w334
              frame False {
                # "These are the remaining states (at the moment the error occured). States can be altered according to business logic."
                # "NOT SHUTTING DOWN"
              }
              frame True {
                # "Developer can decide to alter the states but should be aware that during the shutdown process, there are certain states that must be run for the SMO to properly shut itself (and this process) down. As such, one can add states to perform additional clean-ups, but should append the remaining state to be executed."
                # "SHUTTING DOWN"
                n136 = call <vilib>:"Add State(s) to Queue__jki_lib_state_machine.vi"("State(s) in (\"\")"=w348) -> ("States Out"=w347:string)  [unwired: 14 in]
              }
            }
            n137 = Bundle By Name(cluster=w337, "Core.Last Error.error"=w339) -> (w341:T4)
            n138 = call <vilib>:"Add State(s) to Queue__jki_lib_state_machine.vi"("State(s) in Front (\"\")"=w334, "State(s) in (\"\")"=w345) -> ("States Out"=w344:string)  [unwired: 13 in]
          }
          frame "Macro: Exit" {
            # "Exit Macro\n(This is called once, when the VI exits)"
            n139 = Unbundle By Name(w352) -> ("Core.Close Panel on Exit?"=w359:bool)
            n140 = Bundle By Name(cluster=w352, "Core.Shutdown?"=TRUE) -> (w351:T4)
            n141 = Select(t="UI: Front Panel State >> Close", s=w359, f="") -> (s? t:f=w356:string)
            n142 = call <vilib>:"Add State(s) to Queue__jki_lib_state_machine.vi"("State(s) in (\"\")"=w356, "State(s) at Back (\"\")"="Data: Cleanup\nEvents: Unregister\nProcess: Sync\nExit") -> ("States Out"=w355:string)  [unwired: 13 in]
            n143 = call <vilib>:"Add State(s) to Queue__jki_lib_state_machine.vi"("State(s) in Front (\"\")"=w355, "State(s) in (\"\")"=w362) -> ("States Out"=w361:string)  [unwired: 13 in]
          }
          frame "---------- Process ----------" {
            # "Template Separator\n(You can make a copy of, or modify, this frame)"
            n144 = call <vilib>:"Add State(s) to Queue__jki_lib_state_machine.vi"("State(s) in (\"\")"=w367) -> ("States Out"=w366:string)  [unwired: 14 in]
          }
          frame "Process: Sync" {
            n145 = Unbundle By Name(w375) -> ("SelfRef"=w371:refnum<class "Generator.lvclass">)
            n146 = call <vilib>:"WaitOnProcessSync.vi"("error in (no error)"=w370, "SMO"=w371) -> ("error out"=w369:errorcluster, "Don't run?"=w374:bool)  [unwired: 7 in, 1 out]
            n147 = Select(t="Data: Cleanup\nEvents: Unregister\nExit", s=w374, f="") -> (s? t:f=w368:string)
            n148 = call <vilib>:"Add State(s) to Queue__jki_lib_state_machine.vi"("State(s) in Front (\"\")"=w368, "State(s) in (\"\")"=w378) -> ("States Out"=w377:string)  [unwired: 13 in]
          }
          frame "---------- Events ----------" {
            # "Template Separator\n(You can make a copy of, or modify, this frame)"
            n149 = call <vilib>:"Add State(s) to Queue__jki_lib_state_machine.vi"("State(s) in (\"\")"=w383) -> ("States Out"=w382:string)  [unwired: 14 in]
          }
          frame "Events: Register" {
            n150 = Unbundle By Name(w394) -> ("SelfRef"=w391:refnum<class "Generator.lvclass">)
            n151 = call <vilib>:"GetProtectedEvents.vi"("error in (no error)"=w390, "SMO"=w391) -> ("error out"=w389:errorcluster, "SMO Protected Events"=w393:T16, "SMO out"=w386:refnum<class "Generator.lvclass">)  [unwired: 7 in]
            n152 = call "Generator.GetPrivateEvents.vi"("Generator"=w386) -> ("error out"=w384:errorcluster, "Generator Private Events"=w385:T17)  [unwired: 8 in, 1 out]
            n153 = register-events(w393, w385) -> (reference out=w392:refnum<event-registration>, error out=w388:errorcluster)  [unwired: 2 in]
            n154 = call <vilib>:"Add State(s) to Queue__jki_lib_state_machine.vi"("State(s) in (\"\")"=w396) -> ("States Out"=w395:string)  [unwired: 14 in]
            n155 = Merge Errors(w384, w389, w388) -> (w387:errorcluster)
          }
          frame "Events: Unregister" {
            n156 = Unregister For Events(event registration refnum=w399, error in=w398) -> (error out=w397:errorcluster)
            n157 = call <vilib>:"Clear Errors.vi"("error in (no error)"=w397) -> ()  [unwired: 5 in, 2 out]
            n158 = call <vilib>:"Add State(s) to Queue__jki_lib_state_machine.vi"("State(s) in (\"\")"=w402) -> ("States Out"=w401:string)  [unwired: 14 in]
          }
          frame "--------- Generator ---------" {
            # "Section Separator\n(You can make a copy of, or modify, this frame)"
            n159 = Unbundle By Name(w405) -> ("SelfRef"=w404:refnum<class "Generator.lvclass">)
            n160 = Bundle By Name(cluster=w405, "SelfRef"=w404) -> (w406:T4)
            n161 = call <vilib>:"Add State(s) to Queue__jki_lib_state_machine.vi"("State(s) in (\"\")"=w409) -> ("States Out"=w408:string)  [unwired: 14 in]
          }
          frame "Generator: Generate" {
            # "T: add wfm to queue\nF: generate user event"
            # "Generator: Generate\n(You can make a copy of, or modify, this frame)"
            n162 = Unbundle By Name(w422) -> ("SelfRef"=w421:refnum<class "Generator.lvclass">)
            n163 = call "Generate Waveforms.vi"("error in (no error)"=w425, "Generator.lvclass"=w421) -> ("error out"=w418:errorcluster, "Chart"=→"time (ms)":dbl, "Waveforms out"=w420:T18, "Generator.lvclass"=w419:refnum<class "Generator.lvclass">)  [unwired: 5 in, 1 out]
            n164 = case shown="False" TRUE {
              tunnel: w420 -> [w433 w439]
              tunnel: w419 -> [w434 w438]
              tunnel: w418 -> [w431 w437]
              tunnel: [w432 w436] -> w417
              tunnel: [w430 w435] -> w415
              frame False {
                n165 = call "getWaveforms.vi"("error in (no error)"=w431, "Waveforms"=w433, "Generator in"=w434) -> ("error out"=w430:errorcluster, "Generator out"=w432:refnum<class "Generator.lvclass">)  [unwired: 7 in]
              }
              frame True {
                n166 = call "Generator.AddToQueue.vi"("error in (no error)"=w437, "Waveforms"=w439, "Generator in"=w438) -> ("error out"=w435:errorcluster, "Generator out"=w436:refnum<class "Generator.lvclass">)  [unwired: 7 in]
              }
            }
            n167 = Unbundle By Name(w417) -> ("AO Channels"=w416:T5)
            n168 = call "getAOchannels.vi"("error in (no error)"=w415, "AO Channels"=w416, "Generator in"=w417) -> ("error out"=w414:errorcluster, "Generator out"=w413:refnum<class "Generator.lvclass">)  [unwired: 7 in]
            n169 = Unbundle By Name(w413) -> ("sweep status"=w412:T19)
            n170 = call "getSweepStatus.vi"("error in (no error)"=w414, "sweep status"=w412, "Generator in"=w413) -> ("error out"=w423:errorcluster, "Generator out"=w424:refnum<class "Generator.lvclass">)  [unwired: 7 in]
            n171 = Bundle By Name(cluster=w422, "SelfRef"=w424) -> (w426:T4)
            n172 = call <vilib>:"Add State(s) to Queue__jki_lib_state_machine.vi"("State(s) in (\"\")"=w429) -> ("States Out"=w428:string)  [unwired: 14 in]
          }
        }
      }
    }
    frame Error {
    }
  }
  n173 = call-parent "Process.vi"("error in"=w4, "SMO"=w3) -> ("error out"=w1:errorcluster, "SMO out"=→"Generator out":refnum<class "Generator.lvclass">)  [unwired: 8 in]
  n174 = Merge Errors(w1, w2) -> (→"error out":errorcluster)
